vi "test_data item filter.vi"(7 "data items":string[](array[string]), 8 "error in":errorcluster, 9 "match behavior":T4, 10 "aggregation method":T5=enum."All", 11 "directory":path) -> (0 "error out":errorcluster, 3 "failure info":T1 {"Log Record"."timestamp" format="%<%x %.3X>T"})   [LabVIEW 2018]
uses:
  src/api/extension/filter_interface/Aggregation Method.ctl
  src/api/extension/filter_interface/Match Behavior.ctl
  src/api/logger_class/Failure Information.ctl
  src/api/logger_class/Log Record.ctl
  src/api/logger_class/Internal Log Levels.ctl
  src/api/logger_class/Log Levels.ctl
  src/api/configuration/formatters/format_string_formatter/Format String.lvclass
  C:/Users/Colin/Documents/software_projects/labview/glog/src/api/extension/formatter_interface/Formatter.lvclass
  src/api/configuration/filters/data_item_filter/Data Item.lvclass
  C:/Users/Colin/Documents/software_projects/labview/glog/src/api/extension/filter_interface/Filter.lvclass
  src/api/configuration/handlers/file_handler/File Handler.lvclass
  C:/Users/Colin/Documents/software_projects/labview/glog/src/api/extension/formatting_handler_interface/Formatting Handler.lvclass
  src/api/configuration/filters/data_item_filter/New (Array).vi
  src/api/logger_class/Log (Parts).vi
  src/api/logger_class/Logger.lvclass
  src/api/GLog.lvlib
panel:
  # "Connector Pane"
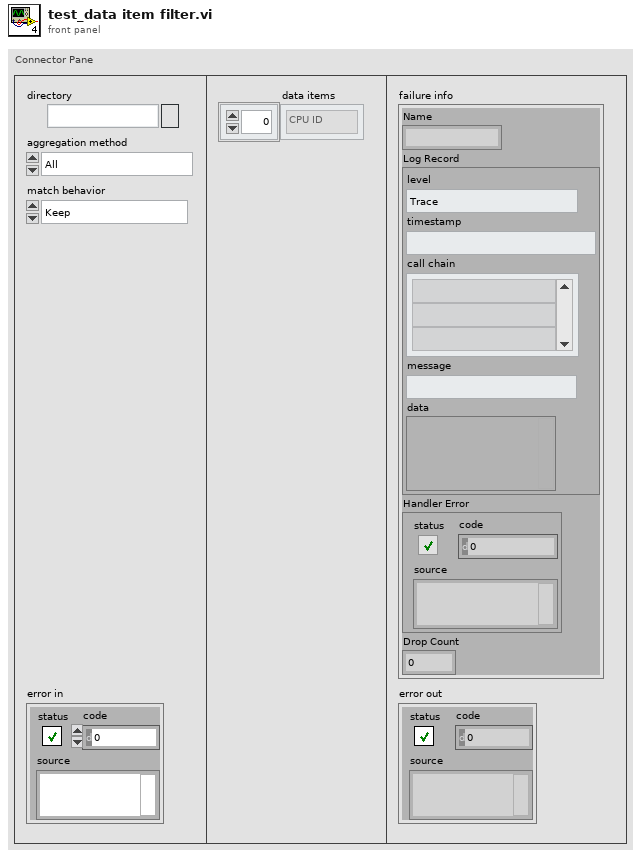
[diagram p1: front panel]
types:
  T1 = typedef "GLog.lvlib/Logger.lvclass/Failure Information.ctl" = cluster{"Name":string, "Log Record":T2, "Handler Error":errorcluster, "Drop Count":u32}
  T2 = typedef "GLog.lvlib/Logger.lvclass/Log Record.ctl" = cluster{"level":T3, "timestamp":timestamp, "call chain":string[], "message":string, "data":variant}
  T3 = typedef "GLog.lvlib/Logger.lvclass/Internal Log Levels.ctl" = enum16{"Trace", "Debug", "Info", "Warning", "Error", "Critical", "Internal"}
  T4 = typedef "GLog.lvlib/Match Behavior.ctl" = enum16{"Keep", "Discard"}
  T5 = typedef "GLog.lvlib/Aggregation Method.ctl" = enum16{"Any", "Only", "All", "None"}
  T6 = typedef "GLog.lvlib/Logger.lvclass/Log Levels.ctl" = enum16{"Trace", "Debug", "Info", "Warning", "Error", "Critical"}
  T7 = cluster{"Iteration":i32, "CPU ID":string, "Machine Name":string, "PID":string}
  T8 = cluster{"Iteration":i32, "CPU ID":string, "Machine Name":string}
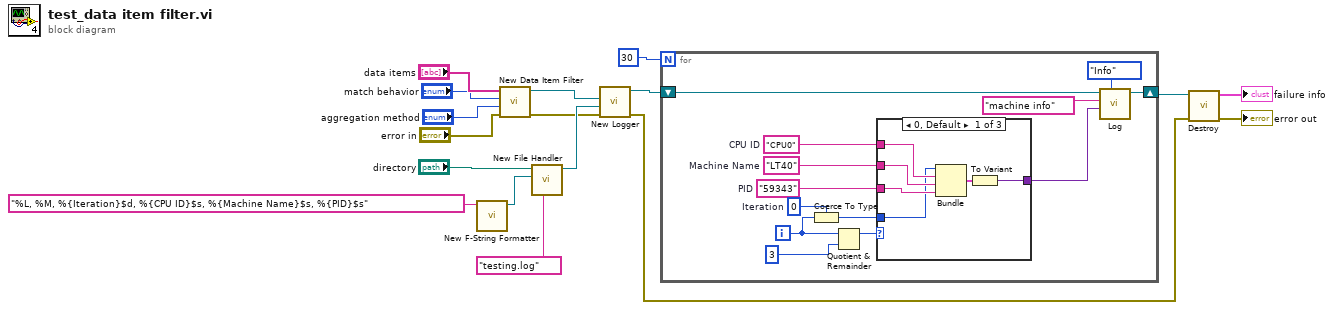
[diagram p0: block diagram]
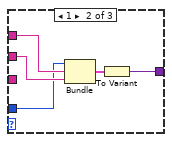
[diagram p2: hidden frame]
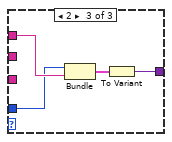
[diagram p3: hidden frame]
diagram:
  n1 = call "New F-String Formatter.vi"("format string (\"%T | %L | %M\")"="%L, %M, %{Iteration}$d, %{CPU ID}$s, %{Machine Name}$s, %{PID}$s" ("format string (\"%T | %L | %M\")")) -> ("new f-string formatter"=w9:refnum<class "Format String.lvclass">)  [unwired: 10 in]
  n2 = call-poly "New Data Item Filter.vi"("error in (no error)"="error in", "aggregation method (all)"="aggregation method", "match behavior (keep)"="match behavior", "data item names"="data items") -> ("error out"=w13:errorcluster, "data item out"=w2:refnum<class "Data Item.lvclass">)  [unwired: 6 in]
  n3 = call "New File Handler.vi"("file name format (\"logfile_%<%Y-%m-%d_%H-%M-%S>T.log\")"="testing.log" ("file name format (\"logfile_%<%Y-%m-%d_%H-%M-%S>T.log\")"), "formatter (JSON)"=w9, "log directory (<app dir>/logs)"="directory") -> ("file handler"=w15:refnum<class "File Handler.lvclass">)  [unwired: 6 in, 2 out]
  n4 = call "New Logger.vi"("error in (no error)"=w13, "log handler (file handler)"=w15, "log filter (none)"=w2) -> ("error out"=w5:errorcluster, "logger"=w10:refnum<class "Logger.lvclass">)  [unwired: 7 in]
  n5 = for {
    N: 30 -> [_]
    shift-right: [w29] -> w6
    shift-left: w10 -> [w30]
    i -> [w21]
    w23 = 0  # Iteration
    w24 = "59343"  # PID
    w25 = "LT40"  # Machine Name
    w26 = "CPU0"  # CPU ID
    n6 = Coerce To Type(0:w21, 1:w23) -> (2:w22:i32)
    n7 = Quotient & Remainder(x=w21, y=3) -> (x-y*floor(x/y)=w27:i32)  [unwired: 1 out]
    n8 = case shown="0, Default" w27 {
      tunnel: w26 -> [w36 w40 w44]
      tunnel: w25 -> [w35 w39 _]
      tunnel: w24 -> [w34 _ _]
      tunnel: [w32 w38 w43] -> w19
      tunnel: w22 -> [w31 w37 w42]
      frame 0, Default {
        n9 = Bundle("Iteration"=w31, "CPU ID"=w36, "Machine Name"=w35, "PID"=w34) -> (w33:T7)  [unwired: 1 in]
        n10 = To Variant(anything=w33) -> (Variant=w32:variant)
      }
      frame 1 {
        n11 = Bundle("Iteration"=w37, "CPU ID"=w40, "Machine Name"=w39) -> (w41:T8)  [unwired: 1 in]
        n12 = To Variant(anything=w41) -> (Variant=w38:variant)
      }
      frame 2 {
        n13 = Bundle("Iteration"=w42, "CPU ID"=w44) -> (w45:cluster{"Iteration":i32, "CPU ID":string})  [unwired: 1 in]
        n14 = To Variant(anything=w45) -> (Variant=w43:variant)
      }
    }
    n15 = call-poly "Log.vi"("log level"=Log_Levels."Info", "data (null)"=w19, "message"="machine info", "logger in"=w30) -> ("logger out"=w29:refnum<class "Logger.lvclass">)  [unwired: 7 in]
  }
  n16 = call "Destroy.vi"("error in (no error)"=w5, "logger in"=w6) -> ("error out"=→"error out":errorcluster, "failure info"=→"failure info":T1)  [unwired: 8 in]
